vi "GDSProject_Create.vi"(1 "ProjectTreePosition(String or Project Item Ref)":variant, 2 "AllowPopUpDilaog(True)":bool=TRUE, 5 "error in (no error)":errorcluster) -> (10 "ProjectItemIn":bool, 14 "Project Refnum":refnum<vi>, 15 "Project Item":refnum<vi>, 17 "App":refnum<vi>, 19 "error out":errorcluster)   [LabVIEW 2020]
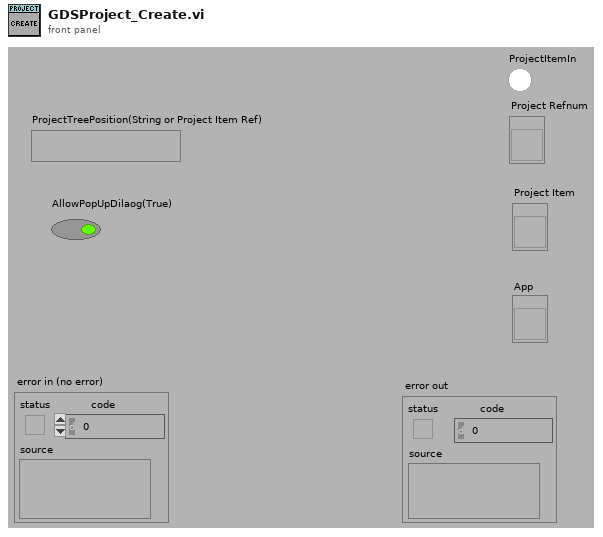
[diagram p1: front panel]
types:
  T1 = enum16{"Left Button", "Center Button", "Right Button", "Window Close"}
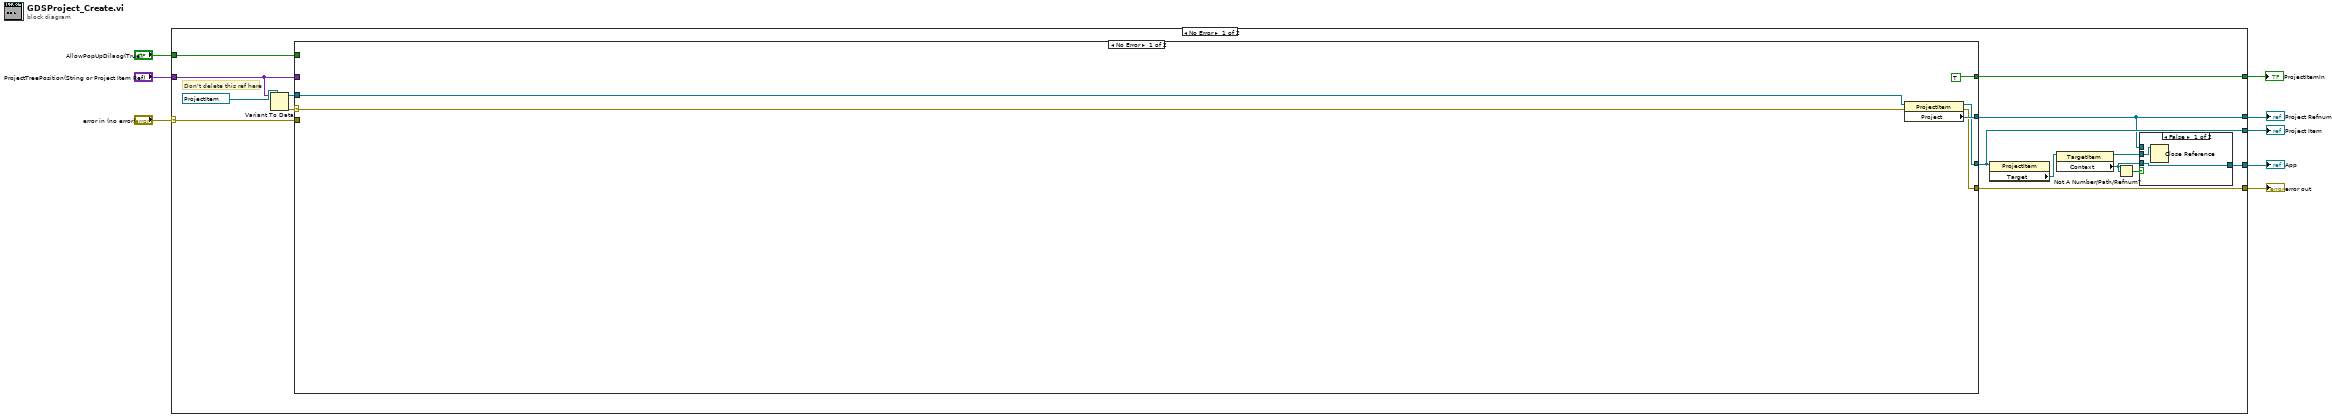
[diagram p0: block diagram]
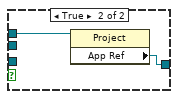
[diagram p2: hidden frame]
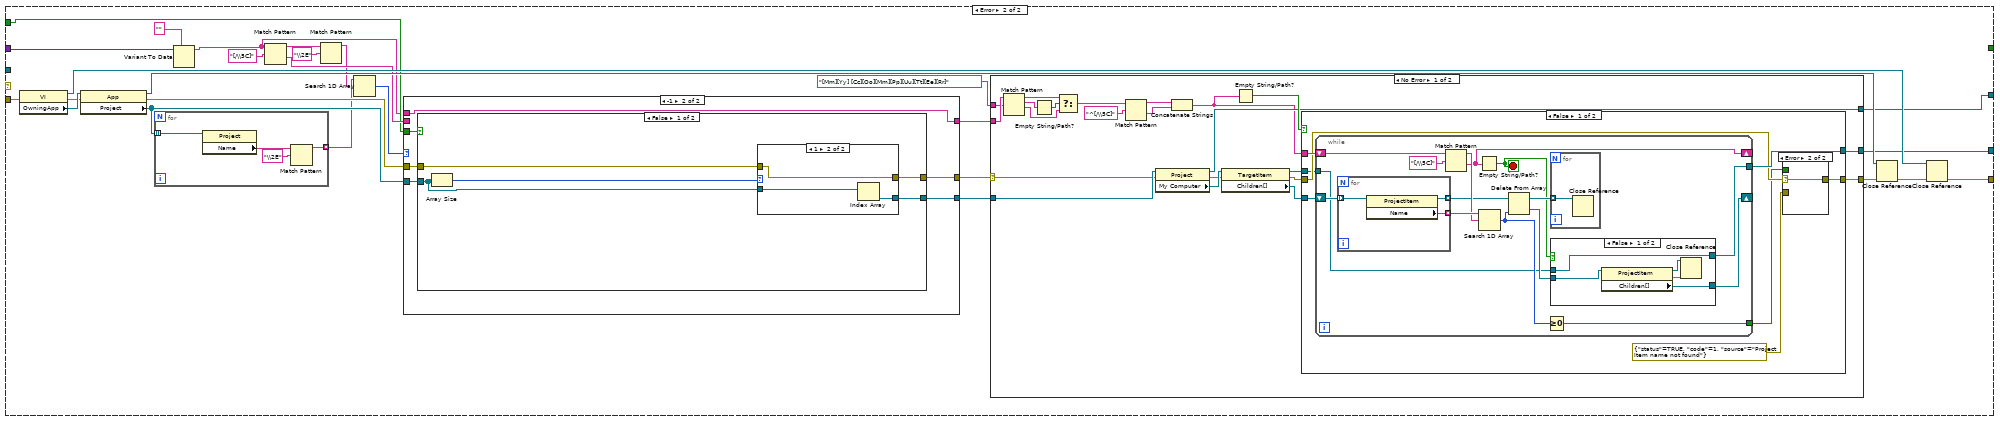
[diagram p3: hidden frame]
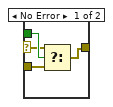
[diagram p4: hidden frame]
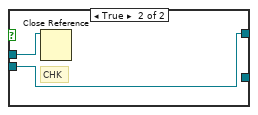
[diagram p5: hidden frame]
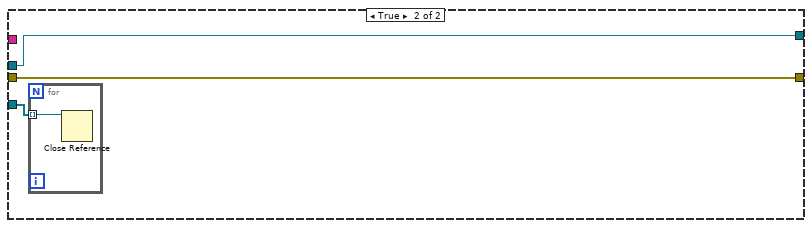
[diagram p6: hidden frame]
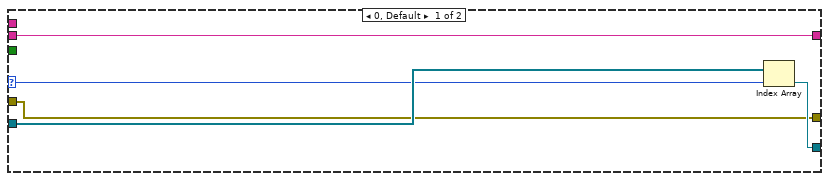
[diagram p8: hidden frame]
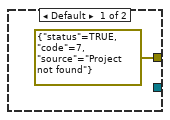
[diagram p9: hidden frame]
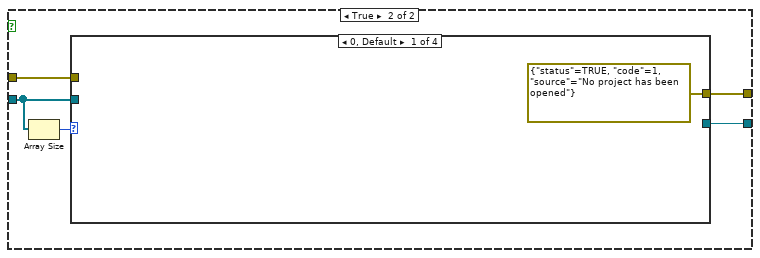
[diagram p10: hidden frame]
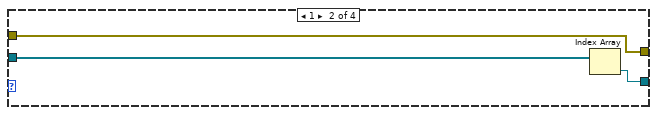
[diagram p11: hidden frame]
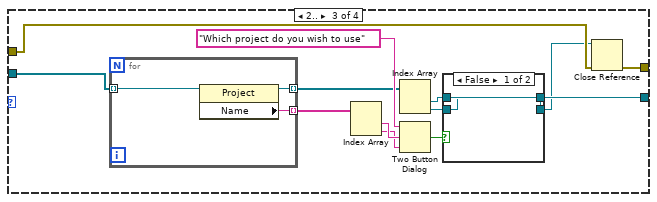
[diagram p12: hidden frame]
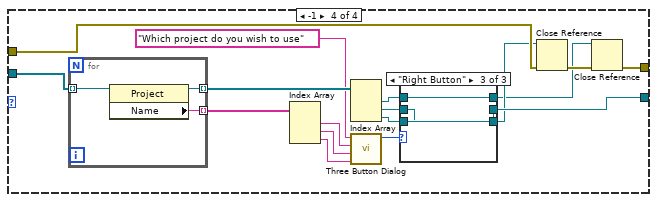
[diagram p14: hidden frame]
diagram:
  n1 = case shown="No Error" "error in (no error)" {
    selector: "error in (no error)" -> [w23 w209]
    tunnel: [w22 w209] -> w7
    tunnel: "ProjectTreePosition(String or Project Item Ref)" -> [w17 _]
    tunnel: [w13 _] -> w5
    tunnel: [w12 _] -> w4
    tunnel: "AllowPopUpDilaog(True)" -> [w21 _]
    tunnel: [w11 _] -> w2
    tunnel: [w9 _] -> w1
    frame No Error {
      # "Don't delete this ref here"
      n2 = Variant To Data(type=refnum<vi> refnum ("Project Item"), Variant=w17) -> (data=w18:refnum<vi>, error out=w19:errorcluster)  [unwired: 1 in]
      n3 = case shown="No Error" w19 {
        selector: w19 -> [w29 _]
        tunnel: w23 -> [_ w59]
        tunnel: [w32 w54] -> w22
        tunnel: [w31 w44] -> w13
        tunnel: [w33 w39] -> w12
        tunnel: w21 -> [_ w38]
        tunnel: w18 -> [w30 _]
        tunnel: w17 -> [_ w36]
        tunnel: [TRUE _] -> w9
        frame No Error {
          n4 = property class="ProjectItem"(reference=w30, error in=w29) -> (reference out=w31:refnum<vi>, error out=w32:errorcluster, "Project"=w33:refnum<vi>)
        }
        frame Error {
          n5 = property class="VI"(error in=w59) -> (reference out=w53:refnum<vi>, error out=w58:errorcluster, "OwningApp"=w60:refnum<vi>)  [unwired: 1 in]
          n6 = property class="App"(reference=w60, error in=w58) -> (reference out=w56:refnum<vi>, error out=w57:errorcluster, "Project"=w52:refnum<vi>[])
          n7 = for {
            tunnel: w52 -> [w208] mode=indexing
            tunnel: [w205] -> w50 mode=indexing
            n8 = property class="Project"(reference=w208) -> ("Name"=w206:string)  [unwired: 1 in, 2 out]
            n9 = Match Pattern(string=w206, regular expression="\\2E") -> (before substring=w205:string)  [unwired: 1 in, 3 out]
          }
          n10 = Variant To Data(type="" ("regular expression"), Variant=w36) -> (data=w34:string)  [unwired: 1 in, 1 out]
          n11 = Match Pattern(string=w34, regular expression="[/\\5C]") -> (before substring=w41:string, after substring=w48:string)  [unwired: 1 in, 2 out]
          n12 = Match Pattern(string=w41, regular expression="\\2E") -> (before substring=w40:string)  [unwired: 1 in, 3 out]
          n13 = Search 1D Array(1D array=w50, element=w40) -> (index of element=w49:i32)  [unwired: 1 in]
          n14 = case shown="-1" w49 {
            selector: w49 -> [w130 _]
            tunnel: [w129 w137] -> w47
            tunnel: w57 -> [w128 w136]
            tunnel: [w128 w135] -> w37
            tunnel: w52 -> [w131 w134]
            tunnel: w34 -> [_ w133]
            tunnel: w48 -> [w127 _]
            tunnel: [w127 w133] -> w46
            tunnel: w38 -> [_ w132]
            frame 0, Default {
              n15 = Index Array(array=w131, index=w130) -> (element=w129:refnum<vi>)
            }
            frame -1 {
              n16 = case shown="False" w132 {
                tunnel: [w138 w151] -> w137
                tunnel: w136 -> [w140 w149]
                tunnel: [w142 w148] -> w135
                tunnel: w134 -> [w139 w147]
                frame False {
                  n17 = Array Size(array=w139) -> (size(s)=w141:i32)
                  n18 = case shown="1" w141 {
                    tunnel: [errorcluster {"status"=TRUE, "code"=7, "source"="Project not found"} ("error out") w146] -> w142
                    tunnel: w140 -> [_ w146]
                    tunnel: w139 -> [_ w145]
                    tunnel: [_ w144] -> w138
                    frame Default {
                    }
                    frame 1 {
                      n19 = Index Array(array=w145) -> (element=w144:refnum<vi>)  [unwired: 1 in]
                    }
                  }
                }
                frame True {
                  n20 = Array Size(array=w147) -> (size(s)=w150:i32)
                  n21 = case shown="0, Default" w150 {
                    tunnel: w147 -> [_ w155 w168 w192]
                    tunnel: [_ w154 w160 w188] -> w151
                    tunnel: w149 -> [_ w153 w158 w186]
                    tunnel: [errorcluster {"status"=TRUE, "code"=1, "source"="No project has been opened"} ("error out") w153 w157 w178] -> w148
                    frame 0, Default {
                    }
                    frame 1 {
                      n22 = Index Array(array=w155) -> (element=w154:refnum<vi>)  [unwired: 1 in]
                    }
                    frame 2.. {
                      n23 = for {
                        tunnel: w168 -> [w175] mode=indexing
                        tunnel: [w174] -> w166 mode=indexing
                        tunnel: [w173] -> w163 mode=indexing
                        n24 = property class="Project"(reference=w175) -> (reference out=w173:refnum<vi>, "Name"=w174:string)  [unwired: 1 in, 1 out]
                      }
                      n25 = Index Array(array=w166) -> (element #1=w165:string, element #2=w164:string)  [unwired: 2 in]
                      n26 = Index Array(array=w163) -> (element #1=w161:refnum<vi>, element #2=w159:refnum<vi>)  [unwired: 2 in]
                      n27 = Two Button Dialog(message="Which project do you wish to use", 1:w164, 2:w165) -> (T button?=w162:bool)
                      n28 = case shown="False" w162 {
                        tunnel: w161 -> [w170 w172]
                        tunnel: [w169 w172] -> w160
                        tunnel: [w170 w171] -> w156
                        tunnel: w159 -> [w169 w171]
                        frame False {
                        }
                        frame True {
                        }
                      }
                      n29 = Close Reference(reference=w156, error in (no error)=w158) -> (error out=w157:errorcluster)
                    }
                    frame -1 {
                      n30 = for {
                        tunnel: w192 -> [w204] mode=indexing
                        tunnel: [w203] -> w191 mode=indexing
                        tunnel: [w202] -> w190 mode=indexing
                        n31 = property class="Project"(reference=w204) -> (reference out=w202:refnum<vi>, "Name"=w203:string)  [unwired: 1 in, 1 out]
                      }
                      n32 = Index Array(array=w191) -> (element #1=w183:string, element #2=w182:string, element #3=w181:string)  [unwired: 3 in]
                      n33 = Index Array(array=w190) -> (element #1=w189:refnum<vi>, element #2=w187:refnum<vi>, element #3=w177:refnum<vi>)  [unwired: 3 in]
                      n34 = call <vilib>:"Three Button Dialog.vi"("Right Button Text (\"Cancel\")"=w181, "Center Button Text (\"No\")"=w182, "Left Button Text (\"Yes\")"=w183, "message"="Which project do you wish to use") -> ("Which Button?"=w180:T1)  [unwired: 7 in]
                      n35 = case shown="\"Right Button\"" w180 {
                        tunnel: w189 -> [w195 w197 w200]
                        tunnel: [w195 w198 w201] -> w188
                        tunnel: [w194 w196 w199] -> w185
                        tunnel: w187 -> [w193 w198 w199]
                        tunnel: w177 -> [w194 w196 w201]
                        tunnel: [w193 w197 w200] -> w176
                        frame "Left Button", Default {
                        }
                        frame "Center Button" {
                        }
                        frame "Right Button" {
                        }
                      }
                      n36 = Close Reference(reference=w185, error in (no error)=w186) -> (error out=w179:errorcluster)
                      n37 = Close Reference(reference=w176, error in (no error)=w179) -> (error out=w178:errorcluster)
                    }
                  }
                }
              }
            }
          }
          n38 = case shown="No Error" w37 {
            selector: w37 -> [w62 w126]
            tunnel: w47 -> [w82 _]
            tunnel: w46 -> [w80 _]
            tunnel: "[Mm][Yy] [Cc][Oo][Mm][Pp][Uu][Tt][Ee][Rr]" ("regular expression") -> [w79 _]
            tunnel: [w73 _] -> w44
            tunnel: [w69 w126] -> w43
            tunnel: [w68 _] -> w39
            frame No Error {
              n39 = Match Pattern(string=w80, regular expression=w79) -> (before substring=w76:string, match substring=w78:string, after substring=w75:string)  [unwired: 1 in, 1 out]
              n40 = Empty String/Path?(string/path=w78) -> (empty?=w77:bool)
              n41 = Select(t=w76, s=w77, f=w75) -> (s? t:f=w67:string)
              n42 = Match Pattern(string=w67, regular expression="^[/\\5C]") -> (before substring=w65:string, after substring=w64:string)  [unwired: 1 in, 2 out]
              n43 = property class="Project"(reference=w82, error in=w62) -> (reference out=w68:refnum<vi>, error out=w72:errorcluster, "My Computer"=w81:refnum<vi>)
              n44 = Concatenate Strings(w65, w64) -> (w63:string)
              n45 = property class="TargetItem"(reference=w81, error in=w72) -> (reference out=w61:refnum<vi>, error out=w70:errorcluster, "Children[]"=w74:refnum<vi>[])
              n46 = Empty String/Path?(string/path=w63) -> (empty?=w71:bool)
              n47 = case shown="False" w71 {
                tunnel: w74 -> [w90 w122]
                tunnel: [w89 w123] -> w73
                tunnel: w63 -> [w88 _]
                tunnel: w70 -> [w87 w124]
                tunnel: [w85 w124] -> w69
                tunnel: w61 -> [w83 w123]
                frame False {
                  n48 = while {
                    shift-right: [w103] -> _
                    shift-left: w90 -> [w110]
                    tunnel: [w102] -> w89
                    shift-right: [w100] -> _
                    shift-left: w88 -> [w101]
                    tunnel: [w98] -> w86
                    tunnel: w83 -> [w96]
                    stop <- w105 stop-if-true
                    n49 = for {
                      tunnel: w110 -> [w121] mode=indexing
                      tunnel: [w120] -> w109 mode=indexing
                      tunnel: [w119] -> w107 mode=indexing
                      n50 = property class="ProjectItem"(reference=w121) -> (reference out=w119:refnum<vi>, "Name"=w120:string)  [unwired: 1 in, 1 out]
                    }
                    n51 = Match Pattern(string=w101, regular expression="[/\\5C]") -> (before substring=w108:string, after substring=w100:string)  [unwired: 1 in, 2 out]
                    n52 = Empty String/Path?(string/path=w100) -> (empty?=w105:bool)
                    n53 = Search 1D Array(1D array=w109, element=w108) -> (index of element=w97:i32)  [unwired: 1 in]
                    n54 = Delete From Array(array=w107, index=w97) -> (deleted portion=w104:refnum<vi>, array with subset deleted=w106:refnum<vi>[])  [unwired: 1 in]
                    n55 = Greater Or Equal To 0?(x=w97) -> (x >= 0?=w98:bool)
                    n56 = for {
                      tunnel: w106 -> [w118] mode=indexing
                      n57 = Close Reference(reference=w118) -> ()  [unwired: 1 in, 1 out]
                    }
                    n58 = case shown="False" w105 {
                      tunnel: w104 -> [w115 w117]
                      tunnel: [w114 _] -> w103
                      tunnel: [w111 w117] -> w102
                      tunnel: w96 -> [w111 w116]
                      frame False {
                        n59 = property class="ProjectItem"(reference=w115) -> (reference out=w112:refnum<vi>, error out=w113:errorcluster, "Children[]"=w114:refnum<vi>[])  [unwired: 1 in]
                        n60 = Close Reference(reference=w112, error in (no error)=w113) -> ()  [unwired: 1 out]
                      }
                      frame True {
                        # "CHK"
                        n61 = Close Reference(reference=w116) -> ()  [unwired: 1 in, 1 out]
                      }
                    }
                  }
                  n62 = case shown="Error" w87 {
                    selector: w87 -> [w93 w95]
                    tunnel: w86 -> [w94 _]
                    tunnel: [w92 w95] -> w85
                    tunnel: errorcluster {"status"=TRUE, "code"=1, "source"="Project Item name not found"} ("f") -> [w91 _]
                    frame No Error {
                      n63 = Select(t=w93, s=w94, f=w91) -> (s? t:f=w92:errorcluster)
                    }
                    frame Error {
                    }
                  }
                }
                frame True {
                  n64 = for {
                    tunnel: w122 -> [w125] mode=indexing
                    n65 = Close Reference(reference=w125) -> ()  [unwired: 1 in, 1 out]
                  }
                }
              }
            }
            frame Error {
            }
          }
          n66 = Close Reference(reference=w56, error in (no error)=w43) -> (error out=w55:errorcluster)
          n67 = Close Reference(reference=w53, error in (no error)=w55) -> (error out=w54:errorcluster)
        }
      }
      n68 = property class="ProjectItem"(reference=w13) -> ("Target"=w16:refnum<vi>)  [unwired: 1 in, 2 out]
      n69 = property class="TargetItem"(reference=w16) -> (reference out=w10:refnum<vi>, "Context"=w14:refnum<vi>)  [unwired: 1 in, 1 out]
      n70 = Not A Number/Path/Refnum?(number/path/refnum=w14) -> (NaN/Path/Refnum?=w15:bool)
      n71 = case shown="False" w15 {
        tunnel: [w25 w27] -> w11
        tunnel: w12 -> [_ w26]
        tunnel: w14 -> [w25 _]
        tunnel: w10 -> [w24 _]
        frame False {
          n72 = Close Reference(reference=w24) -> ()  [unwired: 1 in, 1 out]
        }
        frame True {
          n73 = property class="Project"(reference=w26) -> ("App Ref"=w27:refnum<vi>)  [unwired: 1 in, 2 out]
        }
      }
    }
    frame Error {
    }
  }
  "Project Refnum" <- w4
  "error out" <- w7
  "Project Item" <- w5
  "App" <- w2
  "ProjectItemIn" <- w1
